vi "CANsub_REST_Close.vi"(8 "error in (no error)":errorcluster, 11 "client handle":T1) -> (0 "error out":errorcluster)   [LabVIEW 2021, in "CANsub_Common.lvlib"]
uses:
  CANsub_Common.lvlib
  <vilib>/httpClient/LabVIEWHTTPClient.lvlib
  <vilib>/httpClient/ClientHandle.ctl
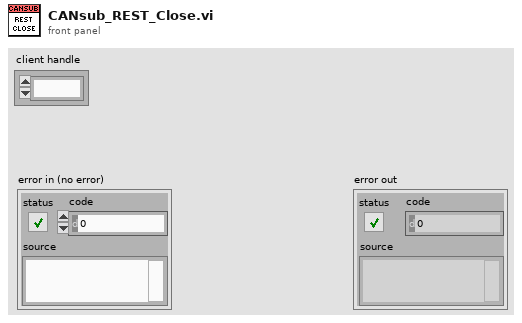
[diagram p1: front panel]
types:
  T1 = typedef "LabVIEWHTTPClient.lvlib/ClientHandle.ctl" = refnum<k1>
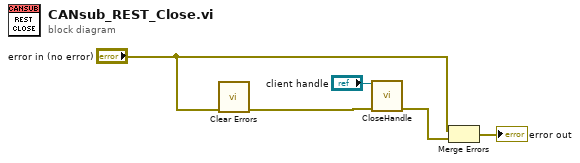
[diagram p0: block diagram]
diagram:
  n1 = call <vilib>:"Clear Errors.vi"("error in (no error)"="error in (no error)") -> ("error out"=w5:errorcluster)  [unwired: 5 in, 1 out]
  n2 = call <vilib>:"CloseHandle.vi"("client handle"="client handle", "error in (no error)"=w5) -> ("error out"=w4:errorcluster)  [unwired: 13 in]
  n3 = Merge Errors("error in (no error)", w4) -> (→"error out":errorcluster)
